vi "scale_graph_units.vi"(7 "error in":errorcluster, 9 "y-units":dbl, 10 "reference in":refnum<vi>) -> (0 "error out":errorcluster, 3 "reference out":refnum<vi>)   [LabVIEW 2025, in "tSNIP.lvlib"]
uses:
  tSNIP.lvlib
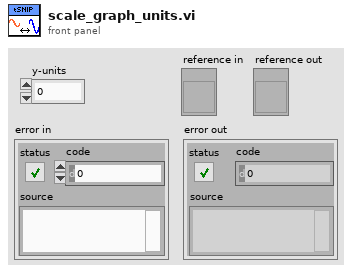
[diagram p1: front panel]
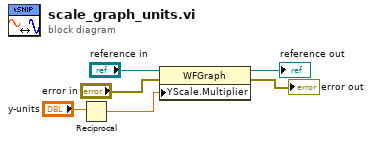
[diagram p0: block diagram]
diagram:
  n1 = Reciprocal(x="y-units") -> (1/x=w1:dbl)
  n2 = property class="WFGraph"(reference="reference in", error in="error in", "YScale.Multiplier"=w1) -> (reference out=→"reference out":refnum<vi>, error out=→"error out":errorcluster)
